vi "C to F convertor.vi"(8 "Temp(C) 4":dbl, 9 "Temp(C) 3":dbl, 10 "Temp(C) 2":dbl, 11 "Temp(C)":dbl) -> (0 "Temp (F) 4":dbl, 1 "Temp (F) 3":dbl, 2 "Temp (F) 2":dbl, 3 "Temp (F)":dbl)   [LabVIEW 2025]
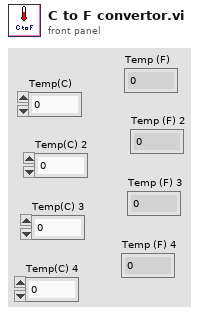
[diagram p1: front panel]
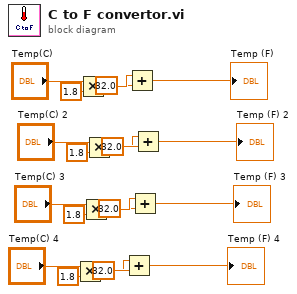
[diagram p0: block diagram]
diagram:
  n1 = Multiply(x="Temp(C) 4", y=1.8) -> (x*y=w3:dbl)
  n2 = Multiply(x="Temp(C)", y=1.8) -> (x*y=w18:dbl)
  n3 = Multiply(x="Temp(C) 3", y=1.8) -> (x*y=w8:dbl)
  n4 = Multiply(x="Temp(C) 2", y=1.8) -> (x*y=w13:dbl)
  n5 = Add(x=w3, y=32.0) -> (x+y=→"Temp (F) 4":dbl)
  n6 = Add(x=w18, y=32.0) -> (x+y=→"Temp (F)":dbl)
  n7 = Add(x=w8, y=32.0) -> (x+y=→"Temp (F) 3":dbl)
  n8 = Add(x=w13, y=32.0) -> (x+y=→"Temp (F) 2":dbl)
